vi "set Attenuation.vi"(8 "error in (no error)":errorcluster, 9 "Auto?":bool, 10 "Attenuation":i32, 11 "Keysight 9020A in":refnum<class "Keysight 9020A.lvclass">) -> (0 "error out":errorcluster, 3 "Keysight 9020A out":refnum<class "Keysight 9020A.lvclass">)   [LabVIEW 2023, in "Spectrum Analyzer.lvlib" / "Keysight 9020A.lvclass"]
uses:
  Keysight 9020A.lvclass
  Keysight 9020A.lvclass/Keysight 9020A.ctl
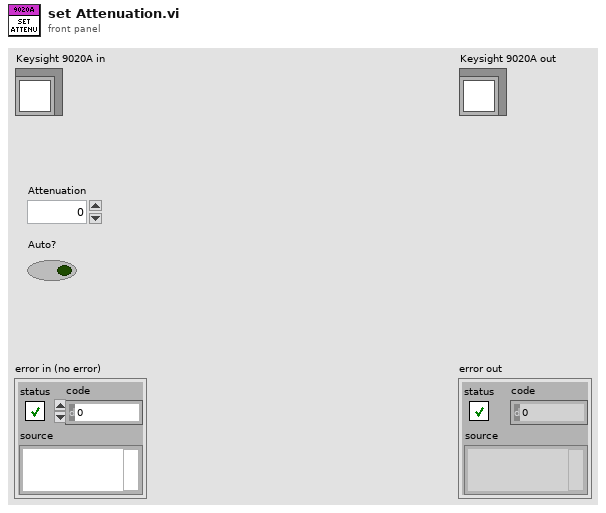
[diagram p1: front panel]
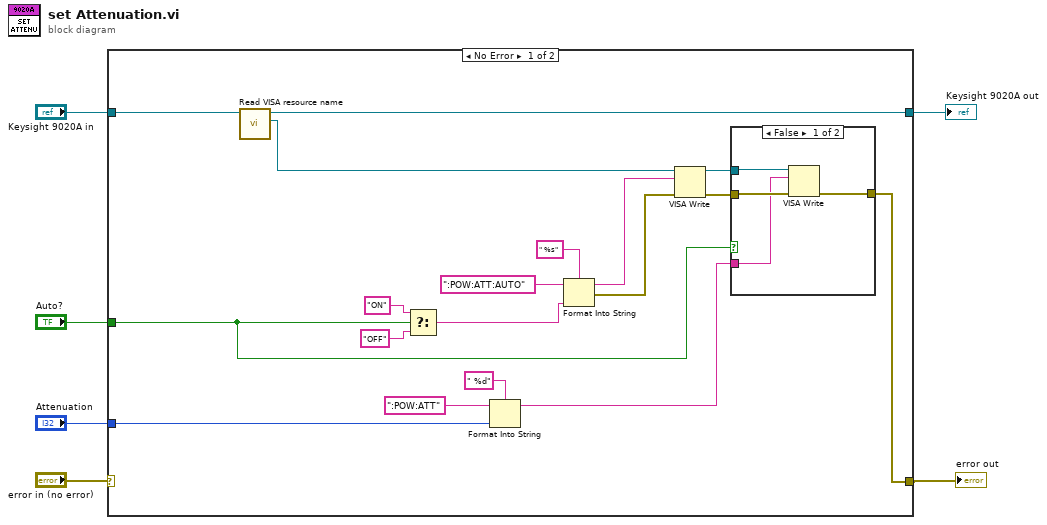
[diagram p0: block diagram]
diagram:
  n1 = case shown="No Error" "error in (no error)" {
    selector: "error in (no error)" -> [_ w30]
    tunnel: "Keysight 9020A in" -> [w14 w31]
    tunnel: [w24 w31] -> w5
    tunnel: [w15 w30] -> w3
    tunnel: "Auto?" -> [w13 _]
    tunnel: "Attenuation" -> [w12 _]
    frame No Error {
      n2 = call "Read VISA resource name.vi"("Keysight 9020A in"=w14) -> ("VISA resource name"=w19:refnum<visa-resource-name>, "Keysight 9020A out"=w24:refnum<class "Keysight 9020A.lvclass">)  [unwired: 8 in, 1 out]
      n3 = Select(t="ON", s=w13, f="OFF") -> (s? t:f=w9:string)
      n4 = Format Into String(format string=" %d", initial string=":POW:ATT", w12) -> (resulting string=w16:string)  [unwired: 1 in, 1 out]
      n5 = Format Into String(format string=" %s", initial string=":POW:ATT:AUTO", w9) -> (resulting string=w8:string, error out=w7:errorcluster)  [unwired: 1 in]
      n6 = VISA Write(VISA resource name=w19, write buffer=w8, error in (no error)=w7) -> (VISA resource name out=w18:refnum<visa-resource-name>, error out=w17:errorcluster)  [unwired: 1 out]
      n7 = case shown="False" w13 {
        tunnel: w18 -> [w28 _]
        tunnel: w17 -> [w27 w29]
        tunnel: w16 -> [w26 _]
        tunnel: [w25 w29] -> w15
        frame False {
          n8 = VISA Write(VISA resource name=w28, write buffer=w26, error in (no error)=w27) -> (error out=w25:errorcluster)  [unwired: 2 out]
        }
        frame True {
        }
      }
    }
    frame Error {
    }
  }
  "error out" <- w3
  "Keysight 9020A out" <- w5
